vi "run_diff.vi"(11 "Command Line":string[](array[string])) -> (2 "stdout | stderr":string, 3 "Return Code":i32)   [LabVIEW 2021, in "Graphical Diff.lvlib"]
uses:
  Graphical Diff.lvlib
  subVIs/Change Type.ctl
  <vilib>/Utility/error.llb/DialogType.ctl
  2984f562-c737-4cc6-a833-ea11c79f98b2.vi
  <vilib>/Utility/error.llb/Error Cluster From Error Code.vi
  <vilib>/Comparison/Equal/Equal Functor/Equal Functor.lvclass
  <vilib>/ErrorRing/Error Ring.xnode
panel:
  out "sandbox":path
  in  "Debug? (F)":bool
  out "Full Report":string
  out "error out":errorcluster
  # "Required by LabVIEWCLI\n(via connector pane)"
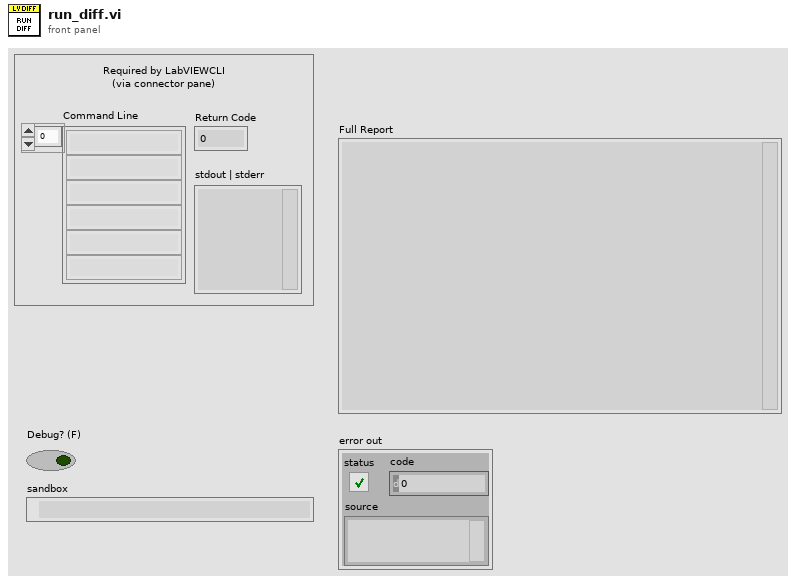
[diagram p1: front panel]
types:
  T1 = typedef "Graphical Diff.lvlib/Change Type.ctl" = enum16{"[undefined]", "Added", "Modified", "Renamed"}
  T2 = cluster{"Change Type":T1, "appended path":path}[]
  T3 = typedef "DialogType.ctl" = u16
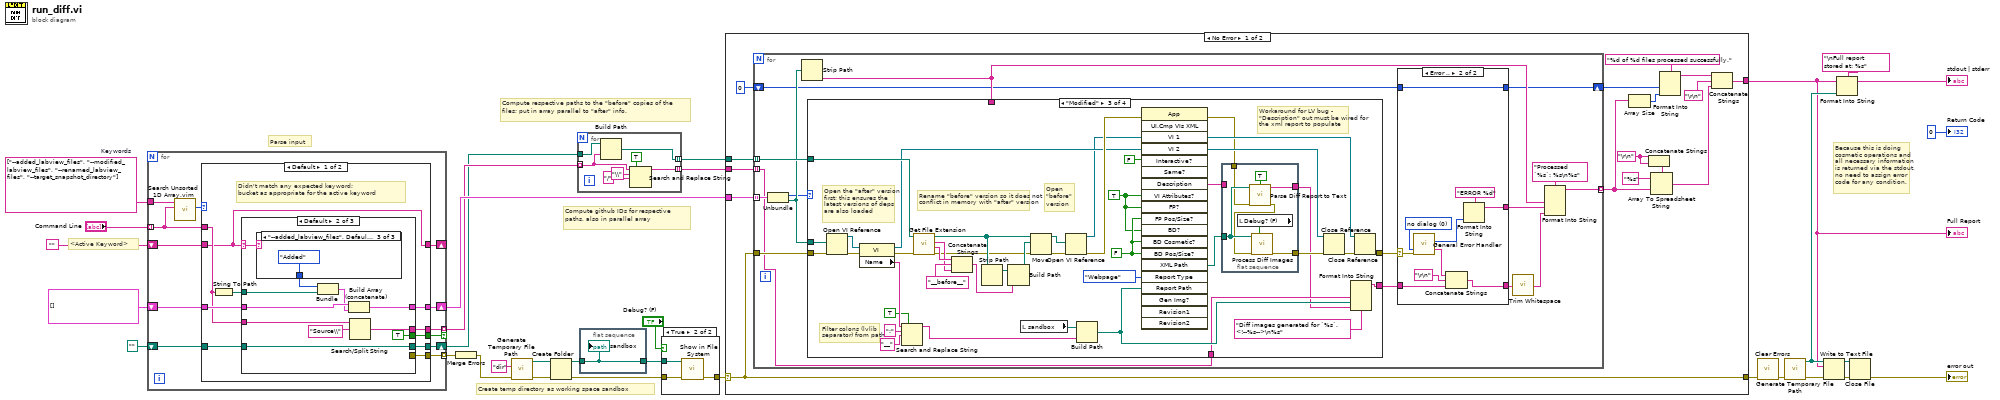
[diagram p0: block diagram]
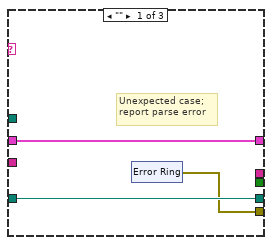
[diagram p3: hidden frame]
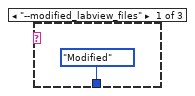
[diagram p4: hidden frame]
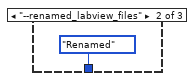
[diagram p5: hidden frame]
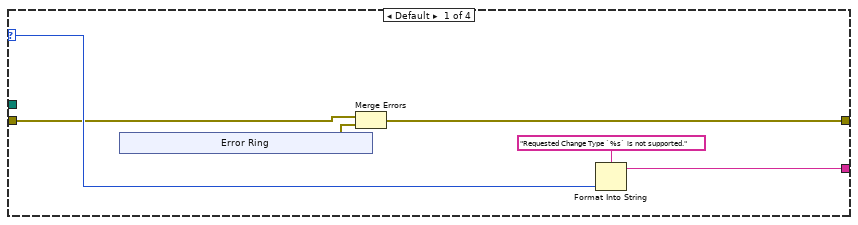
[diagram p8: hidden frame]
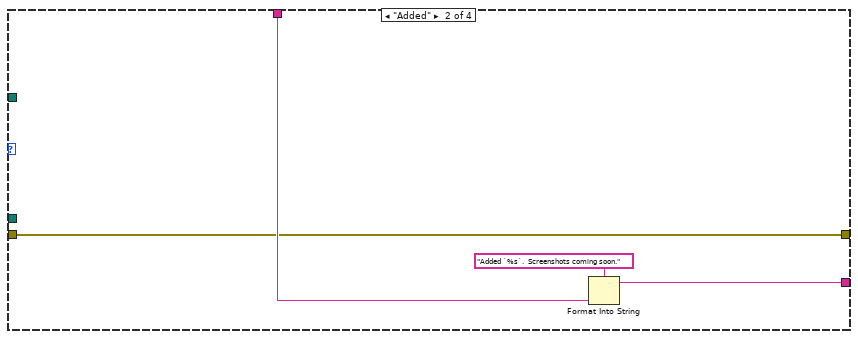
[diagram p9: hidden frame]
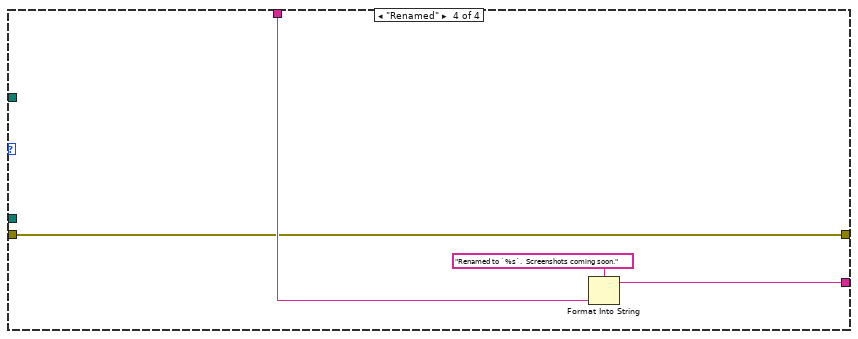
[diagram p10: hidden frame]
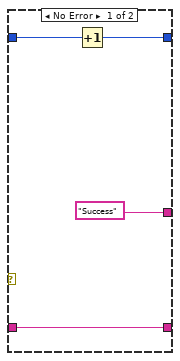
[diagram p11: hidden frame]
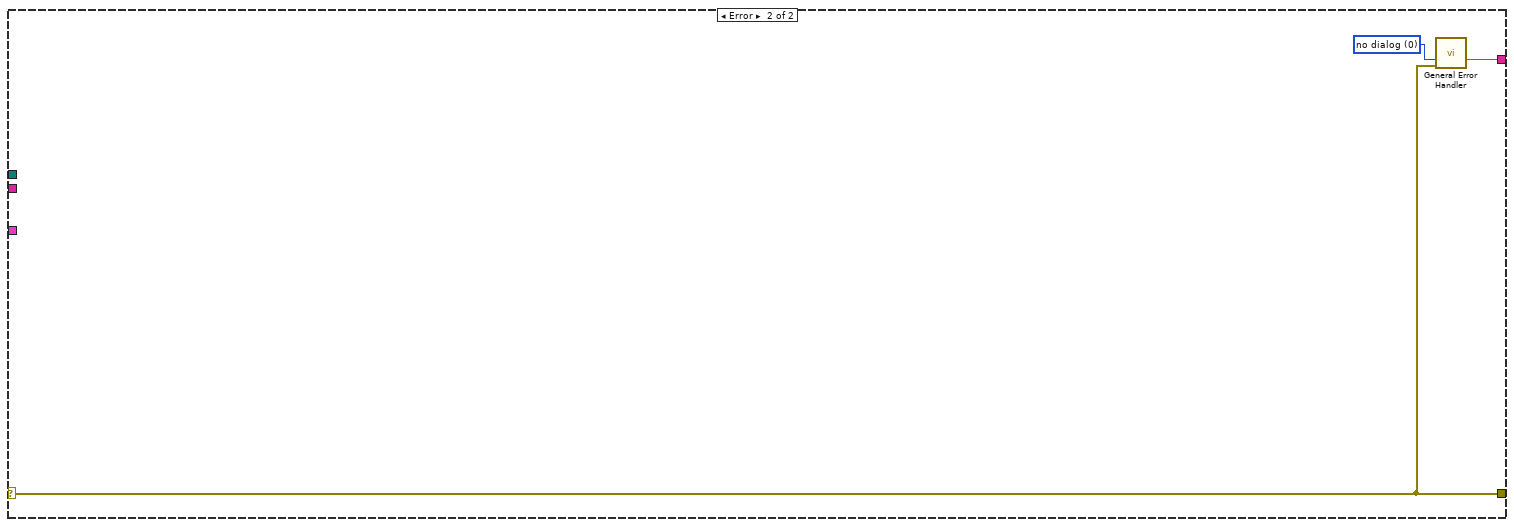
[diagram p12: hidden frame]
diagram:
  w13 = string[] ["--added_labview_files", "--modified_labview_files", "--renamed_labview_files", "--target_snapshot_directory"]  # Keywords
  # "Compute github IDs for respective paths, also in parallel array"
  # "Because this is doing cosmetic operations and all necessary information is returned via the stdout, no need to assign error code for any condition."
  # "<Active Keyword>"
  # "Parse input"
  # "Compute respective paths to the \"before\" copies of the files; put in array parallel to \"after\" info."
  # "Create temp directory as working space sandbox"
  n1 = for {
    tunnel: "Command Line" -> [w34] mode=indexing
    shift-right: [w41] -> w19
    shift-left: T2 [] -> [w42]
    shift-right: [w39] -> w17
    shift-left: path "" -> [w40]
    tunnel: [w38] -> w18 mode=indexing if=w37
    tunnel: [w36] -> w14 mode=indexing
    shift-right: [w32] -> _
    shift-left: "" -> [w33]
    tunnel: w13 -> [w35]
    n2 = call "Search Unsorted 1D Array.vim"("element"=w34, "unsorted 1D array"=w35) -> ("index of element"=w43:i32)  [unwired: 9 in]
    n3 = case shown="Default" w43 {
      tunnel: w42 -> [w49 w79]
      tunnel: [w50 w79] -> w41
      tunnel: w34 -> [w48 w77]
      tunnel: w40 -> [w51 w78]
      tunnel: [w52 w78] -> w39
      tunnel: [w47 _] -> w38
      tunnel: [w46 _] -> w37
      tunnel: [w45 _] -> w36
      tunnel: w33 -> [w44 _]
      tunnel: [w44 w77] -> w32
      frame Default {
        # "Didn't match any expected keyword;\nbucket as appropriate for the active keyword"
        n4 = String To Path(string=w48) -> (path=w53:path)
        n5 = case shown="Default" w44 {
          selector: w44 -> [_ w62 _]
          tunnel: w53 -> [_ w68 w76]
          tunnel: [w56 w71 w76] -> w52
          tunnel: w51 -> [w56 w71 _]
          tunnel: [w55 w69 w75] -> w50
          tunnel: w49 -> [w55 w70 w75]
          tunnel: w48 -> [_ w65 _]
          tunnel: [_ w64 _] -> w47
          tunnel: [_ TRUE _] -> w46
          tunnel: [w54 _ _] -> w45
          frame "" {
            # "Unexpected case; report parse error"
            n6 = xnode "Error Ring"() -> ("error out"=w54:errorcluster)
          }
          frame Default {
            n7 = case shown="\"--added_labview_files\", Default" w62 {
              tunnel: [Change_Type."Modified" ("Change Type") Change_Type."Renamed" ("Change Type") Change_Type."Added" ("Change Type")] -> w61
              frame "--modified_labview_files" {
              }
              frame "--renamed_labview_files" {
              }
              frame "--added_labview_files", Default {
              }
            }
            n8 = Bundle("Change Type"=w61, w68) -> (w67:cluster{"Change Type":T1, path})  [unwired: 1 in]
            n9 = Build Array (concatenate)(w70, w67) -> (w69:T2)
            n10 = Search/Split String(string=w65, search string/char (-)="Source\\") -> (match + rest of string=w64:string)  [unwired: 1 in, 2 out]
          }
          frame "--target_snapshot_directory" {
          }
        }
      }
      frame 0.. {
        # "Matched a known keyword.  Set the \"active\" keyword accordingly."
      }
    }
  }
  n11 = Merge Errors(w14) -> (w15:errorcluster)
  n12 = call <vilib>:"Generate Temporary File Path.vi"("error in (no error)"=w15, "Temporary File Extension (tmp)"="dir") -> ("error out"=w8:errorcluster, "Unique Temporary File Path"=w7:path)  [unwired: 8 in]
  n13 = Create Folder(path (use dialog)=w7, error in=w8) -> (created path=w4:path, error out=w5:errorcluster)  [unwired: 1 in, 1 out]
  n14 = for {
    tunnel: w18 -> [w84] mode=indexing
    tunnel: w17 -> [w86]
    tunnel: [w85] -> w16 mode=indexing
    tunnel: [w80] -> w2 mode=indexing
    n15 = Build Path(base path=w86, name or relative path=w84) -> (appended path=w85:path)
    n16 = Search and Replace String(replace all?=TRUE ("replace all? (F)"), input string=w84, search string="\\", replace string="/" ("replace string (\"\")")) -> (result string=w80:string)  [unwired: 4 in, 3 out]
  }
  n17 = flat-sequence {
    tunnel: w4 -> [w87]
    tunnel: [w87] -> w3
    frame #0 {
      "sandbox" <- w87
    }
  }
  n18 = case shown="True" "Debug? (F)" {
    tunnel: w5 -> [w88 w91]
    tunnel: [w88 w90] -> w23
    tunnel: w3 -> [_ w89]
    frame False {
    }
    frame True {
      n19 = call <vilib>:"Show in File System.vi"("error in (no error)"=w91, "file or directory path"=w89) -> ("error out"=w90:errorcluster)  [unwired: 9 in]
    }
  }
  n20 = case shown="No Error" w23 {
    selector: w23 -> [w106 w202]
    tunnel: w19 -> [w107 _]
    tunnel: [w106 w202] -> w6
    tunnel: [w99 w200] -> w10
    tunnel: w16 -> [w96 _]
    tunnel: w2 -> [w92 _]
    frame No Error {
      w105 = "\r\n"
      n21 = for {
        tunnel: w107 -> [w117] mode=indexing
        tunnel: w106 -> [w123]
        tunnel: [w111] -> w95 mode=indexing
        shift-right: [w109] -> w102
        shift-left: 0 -> [w110]
        tunnel: w96 -> [w116] mode=indexing
        tunnel: w92 -> [w108] mode=indexing
        n22 = Unbundle(w117) -> ("Change Type"=w114:T1, "appended path"=w115:path)
        n23 = Strip Path(path=w115) -> (name=w113:string)  [unwired: 1 out]
        n24 = case shown="\"Modified\"" w114 {
          selector: w114 -> [w128 _ _ _]
          tunnel: w123 -> [w126 w131 w174 w182]
          tunnel: [w127 w132 w150 w183] -> w119
          tunnel: [w125 w131 w153 w182] -> w118
          tunnel: w116 -> [_ _ w162 _]
          tunnel: w115 -> [_ _ w159 _]
          tunnel: w113 -> [_ w133 _ w184]
          tunnel: w108 -> [_ _ w136 _]
          frame Default {
            n25 = xnode "Error Ring"() -> ("error out"=w124:errorcluster)
            n26 = Merge Errors(w126, w124) -> (w125:errorcluster)
            n27 = Format Into String(format string="Requested Change Type `%s` is not supported." ("Control Name"), w128) -> (resulting string=w127:string)  [unwired: 2 in, 1 out]
          }
          frame "Added" {
            n28 = Format Into String(format string="Added `%s`.  Screenshots coming soon.", w133) -> (resulting string=w132:string)  [unwired: 2 in, 1 out]
          }
          frame "Modified" {
            w139 = FALSE
            w138 = TRUE
            # "Workaround for LV bug - \"Description\" out must be wired for the xml report to populate"
            # "Filter colons (lvlib separator) from path"
            # "Rename \"before\" version so it does not conflict in memory with \"after\" version"
            # "Open \"before\" version"
            # "Open the \"after\" version first; this ensures the latest versions of deps are also loaded"
            n29 = Open VI Reference(vi path=w159, error in (no error)=w174) -> (vi reference=w156:refnum<vi>, error out=w158:errorcluster)  [unwired: 4 in]
            n30 = property class="VI"(reference=w156, error in=w158) -> (reference out=w155:refnum<vi>, error out=w157:errorcluster, "Name"=w149:string)
            n31 = Search and Replace String(replace all?=TRUE ("replace all? (F)"), input string=w149, search string=":", replace string="__" ("replace string (\"\")")) -> (result string=w143:string)  [unwired: 4 in, 3 out]
            n32 = call <vilib>:"Get File Extension.vi"("error in (no error)"=w157, "file"=w162) -> ("error out"=w160:errorcluster, "filename without extension"=w168:string, "lowercase file extension"=w167:string, "dup file"=w161:path)  [unwired: 5 in, 1 out]
            n33 = Concatenate Strings(w168, "__before__" ("string"), w167) -> (w166:string)
            n34 = Strip Path(path=w161) -> (stripped path=w171:path)  [unwired: 1 out]
            n35 = Build Path(base path=w171, name or relative path=w166) -> (appended path=w165:path)
            n36 = local read "sandbox"() -> (w141:path)
            n37 = Move(source path=w161, error in=w160, 10:w165) -> (error out=w164:errorcluster, 3:w169:path)  [unwired: 2 in, 1 out]
            n38 = Open VI Reference(vi path=w169, error in (no error)=w164) -> (vi reference=w152:refnum<vi>, error out=w172:errorcluster)  [unwired: 4 in]
            n39 = Build Path(base path=w141, name or relative path=w143) -> (appended path=w137:path)
            n40 = invoke class="App" method="UI.Cmp VIs XML"(error in=w172, "VI 1"=w152, "VI 2"=w155, "Interactive?"=FALSE, "VI Attributes?"=w138, "FP?"=w138, "FP Pos/Size?"=w139, "BD?"=w138, "BD Cosmetic?"=w139, "BD Pos/Size?"=w139, "Report Type"=enum32{"None", "Webpage", "Text", "MS Word"}."Webpage", "Report Path"=w137) -> (error out=w145:errorcluster, "Description"=w142:string, "XML Path"=w140:path)  [unwired: 8 in, 17 out]
            n41 = flat-sequence {
              tunnel: w145 -> [w178]
              tunnel: [w181] -> w144
              tunnel: w142 -> [_]
              tunnel: w140 -> [w179]
              tunnel: [w175] -> w135
              frame #0 {
                n42 = local read "Debug? (F)"() -> (w180:bool)
                n43 = call "Parse Diff Report to Text.vi"("XML Path"=w179, "Attributes only? (F)"=TRUE, "error in"=w178) -> ("change description"=w175:string, "error out"=w177:errorcluster)  [unwired: 11 in]
                n44 = call "Process Diff Images.vi"("Debug? (F)"=w180, "error in (no error)"=w177, "Report path"=w179) -> ("error out"=w181:errorcluster)  [unwired: 8 in]
              }
            }
            n45 = Close Reference(reference=w155, error in (no error)=w144) -> (error out=w154:errorcluster)
            n46 = Format Into String(format string="Diff images generated for `%s`.<!--%s-->\n%s", w136, w137, w135) -> (resulting string=w150:string)  [unwired: 2 in, 1 out]
            n47 = Close Reference(reference=w152, error in (no error)=w154) -> (error out=w153:errorcluster)
          }
          frame "Renamed" {
            n48 = Format Into String(format string="Renamed to `%s`.  Screenshots coming soon.", w184) -> (resulting string=w183:string)  [unwired: 2 in, 1 out]
          }
        }
        n49 = case shown="Error .." w118 {
          selector: w118 -> [_ w198]
          tunnel: ["Success" ("Control Name") w195] -> w121
          tunnel: w119 -> [w189 w194]
          tunnel: [w189 w193] -> w120
          tunnel: w110 -> [w187 w190]
          tunnel: [w186 w190] -> w109
          frame No Error {
            n50 = Increment(x=w187) -> (x+1=w186:i32)
          }
          frame Error {
            w199 = T3 0 items=["no dialog", "OK message", "continue or stop message", "OK message + warnings", "continue/stop + warnings"] ("type of dialog (OK msg:1)")
            n51 = call <vilib>:"General Error Handler.vi"("type of dialog (OK msg:1)"=w199, "error in (no error)"=w198) -> ("code out"=w197:i32, "message"=w192:string)  [unwired: 9 in, 3 out]
            n52 = Concatenate Strings(w192, "\r\n", w194) -> (w193:string)
            n53 = Format Into String(format string="ERROR %d", w197) -> (resulting string=w195:string)  [unwired: 2 in, 1 out]
          }
        }
        n54 = call <vilib>:"Trim Whitespace.vi"("string"=w120) -> ("trimmed string"=w112:string)  [unwired: 1 in]
        n55 = Format Into String(format string="Processed `%s`: %s\n%s" ("Control Name"), w113, w121, w112) -> (resulting string=w111:string)  [unwired: 2 in, 1 out]
      }
      n56 = Array Size(array=w95) -> (size(s)=w101:i32)
      n57 = Concatenate Strings(w105, w105) -> (w98:string)
      n58 = Array To Spreadsheet String(delimiter (Tab)=w98, array=w95, 3:"%s" ("format string")) -> (spreadsheet string=w93:string)
      n59 = Format Into String(format string="%d of %d files processed successfully." ("Control Name"), w102, w101) -> (resulting string=w100:string)  [unwired: 2 in, 1 out]
      n60 = Concatenate Strings(w100, "\r\n", w93) -> (w99:string)
    }
    frame Error {
      w201 = T3 0 items=["no dialog", "OK message", "continue or stop message", "OK message + warnings", "continue/stop + warnings"] ("type of dialog (OK msg:1)")
      n61 = call <vilib>:"General Error Handler.vi"("type of dialog (OK msg:1)"=w201, "error in (no error)"=w202) -> ("message"=w200:string)  [unwired: 9 in, 4 out]
    }
  }
  "Full Report" <- w10
  n62 = call <vilib>:"Clear Errors.vi"("error in (no error)"=w6) -> ("error out"=w31:errorcluster)  [unwired: 5 in, 1 out]
  n63 = call <vilib>:"Generate Temporary File Path.vi"("error in (no error)"=w31) -> ("error out"=w27:errorcluster, "Unique Temporary File Path"=w28:path)  [unwired: 9 in]
  n64 = Write to Text File(file (use dialog)=w28, text=w10, error in=w27) -> (refnum out=w29:refnum<file>, error out=w26:errorcluster)  [unwired: 1 in, 1 out]
  n65 = Format Into String(format string="\nFull report stored at: %s" ("Control Name"), initial string=w10, w28) -> (resulting string=→"stdout | stderr":string)  [unwired: 1 in, 1 out]
  n66 = Close File(refnum=w29, error in=w26) -> (error out=→"error out":errorcluster)  [unwired: 1 out]
  "Return Code" <- 0
